vi "Teleop.vi"(10 "Match Info":T1={"Autonomous Elapsed Seconds"=0.0, "TeleOp Elapsed Seconds"=0.0, "Disabled Elapsed Seconds"=0.0, "Visited Autonomous"=FALSE, "Visited TeleOp"=FALSE, "Visited Disabled"=FALSE, "Autonomous Settings"={"Autonomous Style"=enum."Independent", "VI Refnum"=refnum}}, 11 "Call Context":T2) -> ()   [LabVIEW 2016]
doc: "This VI is called for each TeleOp packet received from the DS where the robot is not disabled. It is often used to read from the joysticks and update I/O or to update setpoints for timed control loops. It should complete and return within 20 milliseconds or it may miss DS packets."
uses:
  <vilib>/Rock Robotics/WPI/DriverStation/WPI_DriverStationDerivedRobotMode.ctl
  <vilib>/Rock Robotics/WPI/DriverStation/WPI_DriverStationMatch Info.ctl
  <vilib>/Rock Robotics/WPI/Utilities/WPI_GetSetVariantRefNum.vi
  Extra/Global_Var-RefNum/Global_Var_Drive.vi
  Extra/Global_Var-RefNum/Global_Var_Other.vi
  ArgosLib/ArgosLib.lvlib
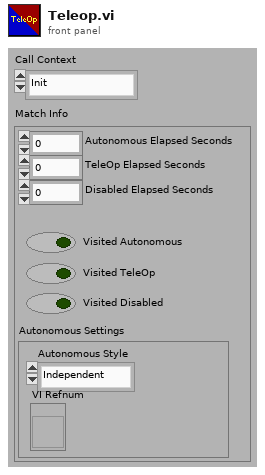
[diagram p1: front panel]
types:
  T1 = typedef "WPI_DriverStationMatch Info.ctl" = cluster{"Autonomous Elapsed Seconds":dbl, "TeleOp Elapsed Seconds":dbl, "Disabled Elapsed Seconds":dbl, "Visited Autonomous":bool, "Visited TeleOp":bool, "Visited Disabled":bool, "Autonomous Settings":cluster{"Autonomous Style":enum16{"Iterative", "Independent"}, "VI Refnum":refnum<vi>}}
  T2 = typedef "WPI_DriverStationDerivedRobotMode.ctl" = enum16{"Init", "Execute", "Stop"}
  T3 = typedef "WPI_JoystickDevRef.ctl" = cluster{"Device":T4}
  T4 = typedef "WPI_JoystickDeviceEnum.ctl" = enum16{"USB 0", "USB 1", "USB 2", "USB 3", "USB 4", "USB 5"}
  T5 = cluster{"Left_Trigger":dbl, "Right_Trigger ":dbl, "Left_X":dbl, "Left_Y":dbl, "Right_X":dbl, "Right_Y":dbl}
  T6 = cluster{"A":bool, "B":bool, "X":bool, " Y":bool, "LB":bool, " RB":bool, "Left_Thumb_Button":bool, "Right_Thumb_Button":bool, "Back":bool, "Start":bool}
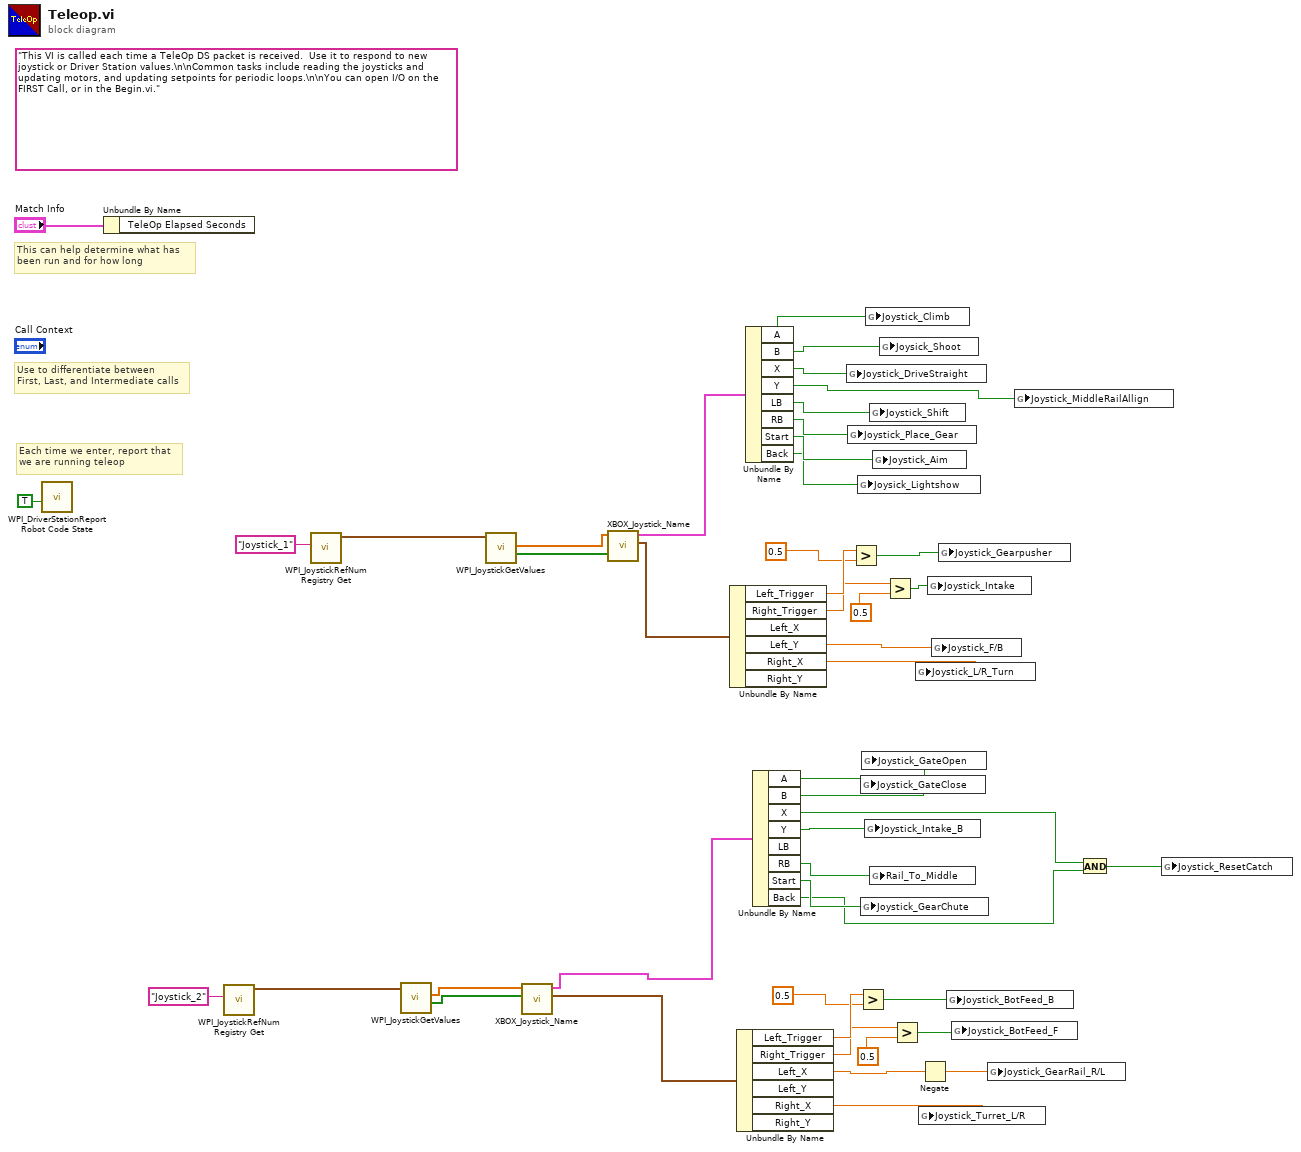
[diagram p0: block diagram]
diagram:
  (unwired) "This VI is called each time a TeleOp DS packet is received.  Use it to respond to new joystick or Driver Station values.\n\nCommon tasks include reading the joysticks and updating motors, and updating setpoints for periodic loops.\n\nYou can open I/O on the FIRST Call, or in the Begin.vi."
  # "Each time we enter, report that\nwe are running teleop"
  # "Use to differentiate between\nFirst, Last, and Intermediate calls"
  # "This can help determine what has\nbeen run and for how long"
  n1 = call <vilib>:"WPI_DriverStationReport Robot Code State.vi"("TeleOp"=TRUE ("Autonomous")) -> ()  [unwired: 10 in, 1 out]
  n2 = Unbundle By Name("Match Info") -> ()  [unwired: 1 out]
  n3 = call <vilib>:"WPI_JoystickRefNum Registry Get.vi"("refnum name"="Joystick_2") -> ("JoystickDevRef"=w42:T3)  [unwired: 9 in, 1 out]
  n4 = call <vilib>:"WPI_JoystickRefNum Registry Get.vi"("refnum name"="Joystick_1") -> ("JoystickDevRef"=w43:T3)  [unwired: 9 in, 1 out]
  n5 = call <vilib>:"WPI_JoystickGetValues.vi"("JoystickDevRef"=w42) -> ("Buttons"=w38:bool[], "Axes"=w39:dbl[])  [unwired: 6 in, 3 out]
  n6 = call <vilib>:"WPI_JoystickGetValues.vi"("JoystickDevRef"=w43) -> ("Buttons"=w41:bool[], "Axes"=w40:dbl[])  [unwired: 6 in, 3 out]
  n7 = call "XBOX_Joystick_Name.vi"("Buttons"=w38, "Axes"=w39) -> ("Named_Axes"=w25:T5, "Named_Buttons"=w26:T6)  [unwired: 8 in]
  n8 = call "XBOX_Joystick_Name.vi"("Buttons"=w41, "Axes"=w40) -> ("Named_Axes"=w36:T5, "Named_Buttons"=w37:T6)  [unwired: 8 in]
  n9 = Unbundle By Name(w36) -> ("Left_Trigger"=w35:dbl, "Right_Trigger"=w33:dbl, "Left_Y"=w19:dbl, "Right_X"=w18:dbl)  [unwired: 2 out]
  n10 = Unbundle By Name(w25) -> ("Left_Trigger"=w30:dbl, "Right_Trigger"=w28:dbl, "Left_X"=w11:dbl, "Right_X"=w12:dbl)  [unwired: 2 out]
  n11 = Unbundle By Name(w37) -> ("A"=w31:bool, "B"=w4:bool, "X"=w9:bool, "Y"=w3:bool, "LB"=w24:bool, "RB"=w5:bool, "Start"=w23:bool, "Back"=w22:bool)
  n12 = Unbundle By Name(w26) -> ("A"=w17:bool, "B"=w16:bool, "X"=w8:bool, "Y"=w15:bool, "RB"=w2:bool, "Start"=w10:bool, "Back"=w7:bool)  [unwired: 1 out]
  n13 = global write "Global_Var_Drive.vi" "Joystick_DriveStraight"(w9) -> ()
  n14 = global write "Global_Var_Drive.vi" "Joystick_Place_Gear"(w5) -> ()
  n15 = Greater?(x=w35, y=0.5) -> (0:w21:bool)
  n16 = global write "Global_Var_Drive.vi" "Joysick_Lightshow"(w22) -> ()
  n17 = Greater?(x=w30, y=0.5) -> (0:w14:bool)
  n18 = global write "Global_Var_Drive.vi" "Joystick_GateClose"(w16) -> ()
  n19 = global write "Global_Var_Drive.vi" "Joystick_GearChute"(w10) -> ()
  n20 = global write "Global_Var_Drive.vi" "Joystick_GateOpen"(w17) -> ()
  n21 = global write "Global_Var_Drive.vi" "Joystick_Intake_B"(w15) -> ()
  n22 = global write "Global_Var_Drive.vi" "Joystick_Climb"(w31) -> ()
  n23 = global write "Global_Var_Drive.vi" "Joystick_Shift"(w24) -> ()
  n24 = global write "Global_Var_Other.vi" "Rail_To_Middle"(w2) -> ()
  n25 = global write "Global_Var_Drive.vi" "Joystick_Aim"(w23) -> ()
  n26 = global write "Global_Var_Drive.vi" "Joysick_Shoot"(w4) -> ()
  n27 = Greater?(x=w33, y=0.5) -> (0:w20:bool)
  n28 = Greater?(x=w28, y=0.5) -> (0:w13:bool)
  n29 = global write "Global_Var_Drive.vi" "Joystick_L/R_Turn"(w18) -> ()
  n30 = global write "Global_Var_Drive.vi" "Joystick_Turret_L/R"(w12) -> ()
  n31 = Negate(x=w11) -> (-x=w1:dbl)
  n32 = global write "Global_Var_Drive.vi" "Joystick_Intake"(w20) -> ()
  n33 = global write "Global_Var_Drive.vi" "Joystick_F/B"(w19) -> ()
  n34 = global write "Global_Var_Drive.vi" "Joystick_Gearpusher"(w21) -> ()
  n35 = global write "Global_Var_Drive.vi" "Joystick_BotFeed_B"(w14) -> ()
  n36 = global write "Global_Var_Drive.vi" "Joystick_BotFeed_F"(w13) -> ()
  n37 = global write "Global_Var_Drive.vi" "Joystick_GearRail_R/L"(w1) -> ()
  n38 = global write "Global_Var_Drive.vi" "Joystick_MiddleRailAllign"(w3) -> ()
  n39 = And(x=w8, y=w7) -> (x .and. y?=w6:bool)
  n40 = global write "Global_Var_Drive.vi" "Joystick_ResetCatch"(w6) -> ()
